vi "Scale Data.vi"(8 "error in":errorcluster, 10 "Raw Graph Data":T10, 11 "Channel Settings in":T1) -> (0 "error out":errorcluster, 2 "Scaled Graph Data":T10, 3 "Channel Settings out":T1)   [LabVIEW 2021, in "Acquisition.lvlib"]
doc: "Use the Calibration Information from 'Channel Settings' to scale the 'Raw Graph Data' and return it in 'Scaled Graph Data'."
uses:
  Acquisition.lvlib
  Acquired Data.ctl
  Hardware Configuration.ctl
  Channel Settings.ctl
  IO Device.ctl
  Sensor Type.ctl
  Interval Timer/Repeat Interval.ctl
  Interval Timer/Interval Length.ctl
  Interval Timer/Interval Token.ctl
  IO Context.ctl
  IO API.ctl
  Interval Timer/Interval Timer.lvlib
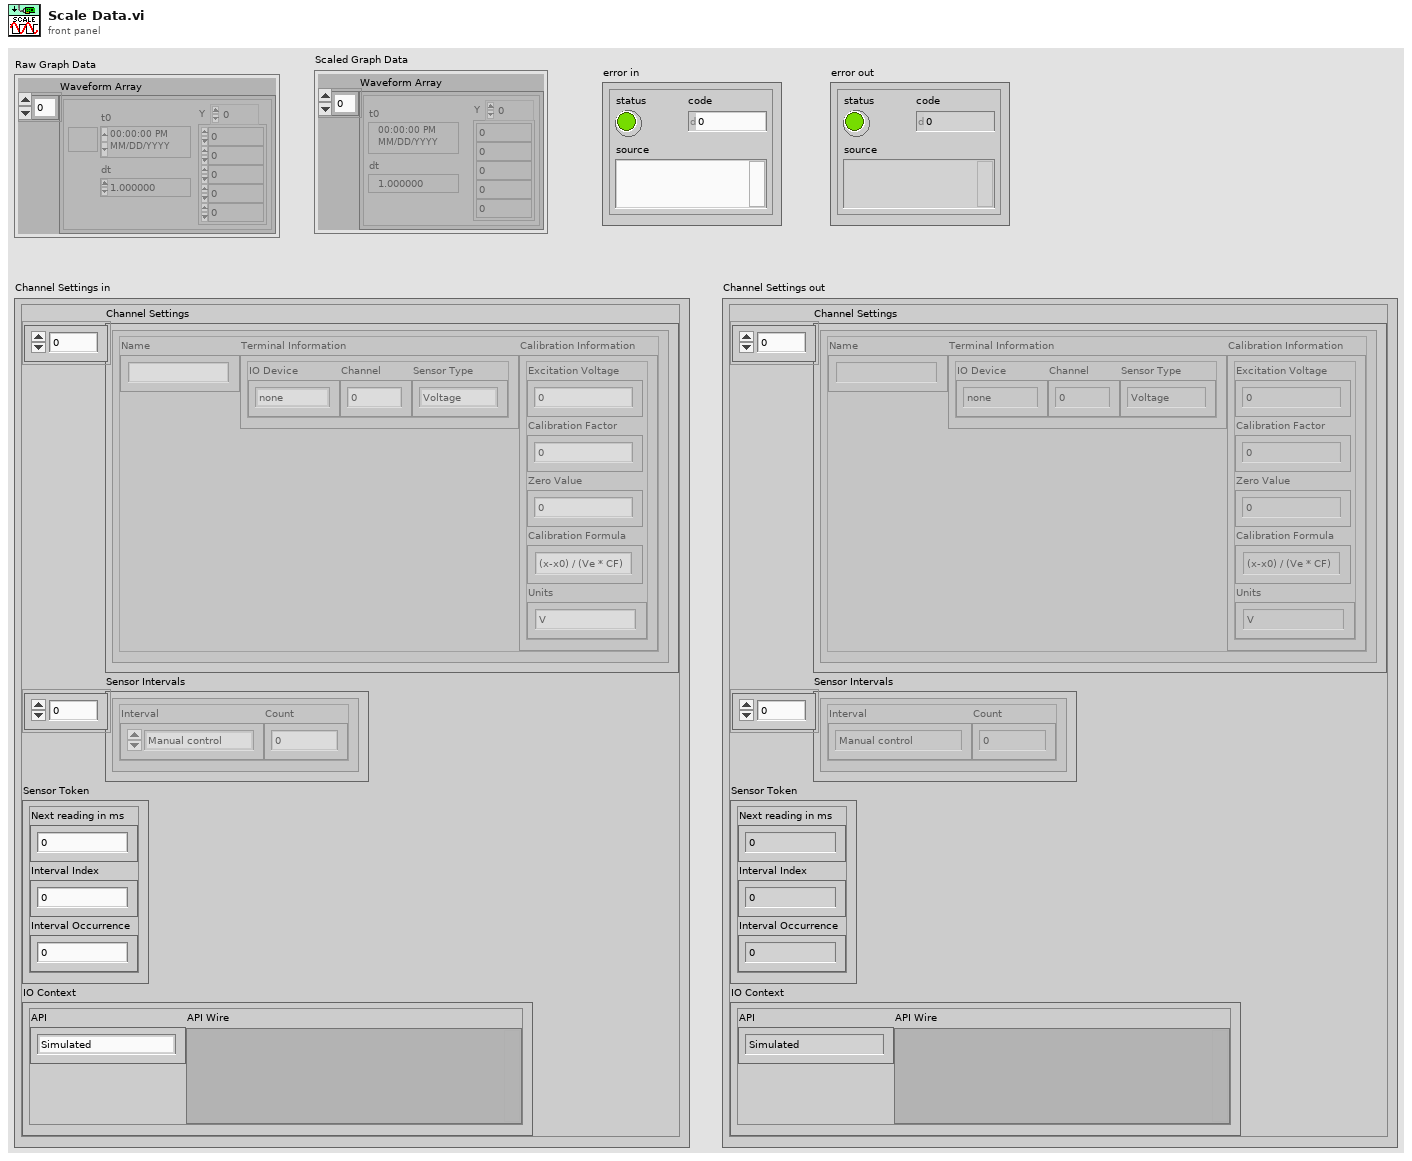
[diagram p1: front panel]
types:
  T1 = typedef "Acquisition.lvlib/Hardware Configuration.ctl" = cluster{"Channel Settings":T2[], "Sensor Intervals":T5[], "Sensor Token":T7, "IO Context":T8}
  T2 = typedef "Acquisition.lvlib/Channel Settings.ctl" = cluster{"Name":string, "Terminal Information":cluster{"IO Device":T3, "Channel":i32, "Sensor Type":T4}, "Calibration Information":cluster{"Excitation Voltage":dbl, "Calibration Factor":dbl, "Zero Value":dbl, "Calibration Formula":string, "Units":string}}
  T3 = typedef "Acquisition.lvlib/IO Device.ctl" = enum16{"none", "9219", "9401"}
  T4 = typedef "Acquisition.lvlib/Sensor Type.ctl" = enum16{"Voltage", "Load", "Pressure", "Encoder"}
  T5 = typedef "Interval Timer.lvlib/Repeat Interval.ctl" = cluster{"Interval":T6, "Count":i32}
  T6 = typedef "Interval Timer.lvlib/Interval Length.ctl" = enum16{"Manual control", "1 second", "10 seconds", "30 seconds", "60 seconds", "600 seconds", "1200 seconds", "3600 seconds"}
  T7 = typedef "Interval Timer.lvlib/Interval Token.ctl" = cluster{"Next reading in ms":u32, "Interval Index":i32, "Interval Occurrence":i32}
  T8 = typedef "Acquisition.lvlib/IO Context.ctl" = cluster{"API":T9, "API Wire":variant}
  T9 = typedef "Acquisition.lvlib/IO API.ctl" = enum16{"Simulated", "DAQmx"}
  T10 = typedef "Acquisition.lvlib/Acquired Data.ctl" = cluster{"Waveform Array":waveform(dbl)[]}
  T11 = cluster{"Excitation Voltage":dbl, "Calibration Factor":dbl, "Zero Value":dbl, "Calibration Formula":string, "Units":string}
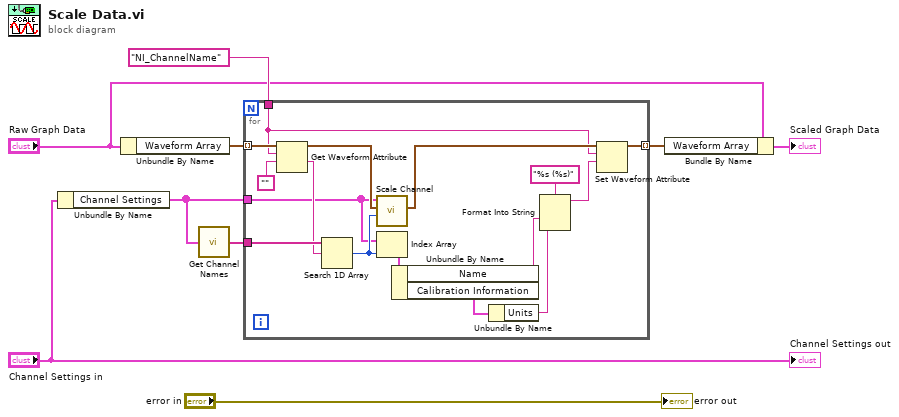
[diagram p0: block diagram]
diagram:
  n1 = Unbundle By Name("Channel Settings in") -> ("Channel Settings"=w2:T2[])
  n2 = Unbundle By Name("Raw Graph Data") -> ("Waveform Array"=w9:waveform(dbl)[])
  n3 = call "Get Channel Names.vi"("Channel Settings"=w2) -> ("Channel Names"=w5:string[])
  n4 = for {
    tunnel: w9 -> [w25] mode=indexing
    tunnel: "NI_ChannelName" ("name") -> [w18]
    tunnel: w5 -> [w23]
    tunnel: w2 -> [w14]
    tunnel: [w19] -> w4 mode=indexing
    n5 = Get Waveform Attribute(5:"", 6:w18, 7:w25) -> (1:w22:string, 3:w21:waveform(dbl))  [unwired: 1 in, 2 out]
    n6 = Search 1D Array(1D array=w23, element=w22) -> (index of element=w15:i32)  [unwired: 1 in]
    n7 = call "Scale Channel.vi"("channel to scale"=w15, "Waveform in"=w21, "Channel Settings"=w14) -> ("Scaled waveform"=w20:waveform(dbl))  [unwired: 6 in, 2 out]
    n8 = Index Array(array=w14, index=w15) -> (element=w13:T2)
    n9 = Unbundle By Name(w13) -> ("Name"=w12:string, "Calibration Information"=w11:T11)
    n10 = Unbundle By Name(w11) -> ("Units"=w10:string)
    n11 = Format Into String(format string="%s (%s)", w12, w10) -> (resulting string=w16:string)  [unwired: 2 in, 1 out]
    n12 = Set Waveform Attribute(5:w16, 6:w18, 7:w20) -> (3:w19:waveform(dbl))  [unwired: 1 in, 2 out]
  }
  n13 = Bundle By Name(cluster="Raw Graph Data", "Waveform Array"=w4) -> (→"Scaled Graph Data":T10)
  "Channel Settings out" <- "Channel Settings in"
  "error out" <- "error in"
